vi "Event WaitForCompletion.vi"(8 "error in (no error)":errorcluster, 11 "Event in":refnum<class "Event.lvclass">) -> (0 "error out":errorcluster, 3 "Event out":refnum<class "Event.lvclass">)   [LabVIEW 2020, in "OpenLvVision_OpenCv.lvlib" / "Cuda.lvlib" / "Event.lvclass"]
doc: "Blocks the calling CPU thread until the event has triggered."
uses:
  Event.lvclass
  C:/Users/lukas/Downloads/OpenLvVision_OpenCv/SourceCode/LabView/OpenLvVision_OpenCv/_LvHelpers/EdvrObject/EdvrObject.lvclass
  _LvHelpers/EdvrObject/EdvrObject.lvclass/EdvrObject.ctl
  OpenLvVision_OpenCv.lvlib
  _LvHelpers/EdvrObject/EdvrObject.lvclass
  <vilib>/Utility/error.llb/Error Cluster From Error Code.vi
  <vilib>/ErrorRing/Error Ring.xnode
  Dlls/OlvOpenCvWrapper.dll
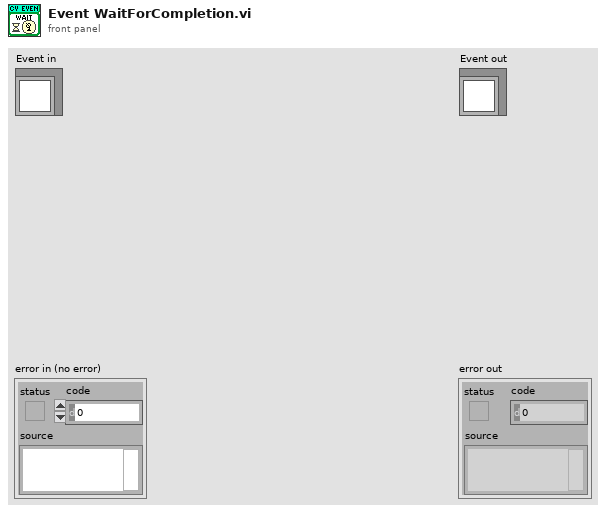
[diagram p1: front panel]
types:
  T1 = typedef "OpenLvVision_OpenCv.lvlib/EdvrObject.lvclass/Edvr.ctl" = refnum<data-value>
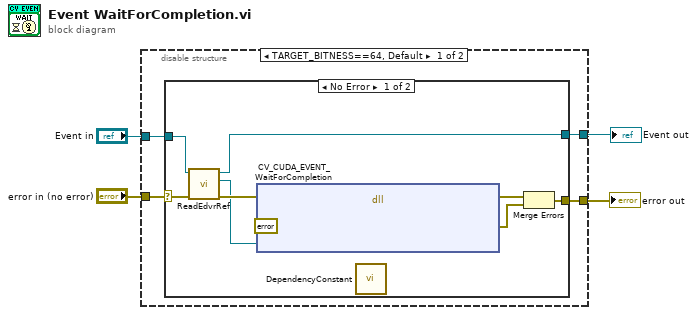
[diagram p0: block diagram]
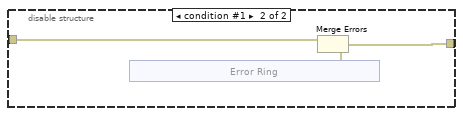
[diagram p3: hidden frame]
diagram:
  n1 = disable-structure shown="TARGET_BITNESS==64, Default" {
    disable-tunnel: "error in (no error)" -> [w5 w21]
    disable-tunnel: [w8 w22] -> w4
    disable-tunnel: [w7 _] -> w3
    disable-tunnel: "Event in" -> [w6 _]
    frame condition #0 (active) {
      n2 = case shown="No Error" w5 {
        selector: w5 -> [w11 w19]
        tunnel: [w13 w19] -> w8
        tunnel: [w14 w18] -> w7
        tunnel: w6 -> [w12 w18]
        frame No Error {
          n3 = call "ReadEdvrRef.vi"("error in (no error)"=w11, "EdvrObject in"=w12) -> ("error out"=w16:errorcluster, "Edvr"=w15:T1, "EdvrObject out"=w14:refnum<class "Event.lvclass">)  [unwired: 7 in]
          n4 = dll-call lib="C:/Users/lukas/Downloads/OpenLvVision_OpenCv/SourceCode/LabView/OpenLvVision_OpenCv/Dlls/OlvOpenCvWrapper.dll" fn="CV_CUDA_EVENT_WaitForCompletion"(error in=w16, "Error"=errorcluster {"status"=FALSE, "code"=0, "source"=""} ("error out"), "eventEdvrRef"=w15) -> (error out=w9:errorcluster, "Error"=w10:errorcluster)  [unwired: 4 in, 1 out]
          n5 = call "DependencyConstant.vi"() -> ()  [unwired: 12 in]
          n6 = Merge Errors(w9, w10) -> (w13:errorcluster)
        }
        frame Error {
        }
      }
    }
    frame condition #1 {
      n7 = xnode "Error Ring"() -> ("error out"=w20:errorcluster)
      n8 = Merge Errors(w21, w20) -> (w22:errorcluster)
    }
  }
  "error out" <- w4
  "Event out" <- w3
